vi "Init Plot Toolbar.vi"(7 "panel mode":T1, 8 "error in (no error)":errorcluster, 11 "Refs":T2) -> (0 "error out":errorcluster, 3 "Refs (dup)":T2)   [LabVIEW 2021, in "RocketPlot.lvlib"]
uses:
  RocketPlot.lvlib
  TypeDefs/Plot UI references.ctl
  <userlib>/bjustice/TipStripOOPanel/Classes/TipPanelHandle/TipPanelHandle.lvclass
  TypeDefs/Plot top row.ctl
  Classes/RocketPlotHandle/RocketPlotHandle.lvclass
  TypeDefs/panel mode.ctl
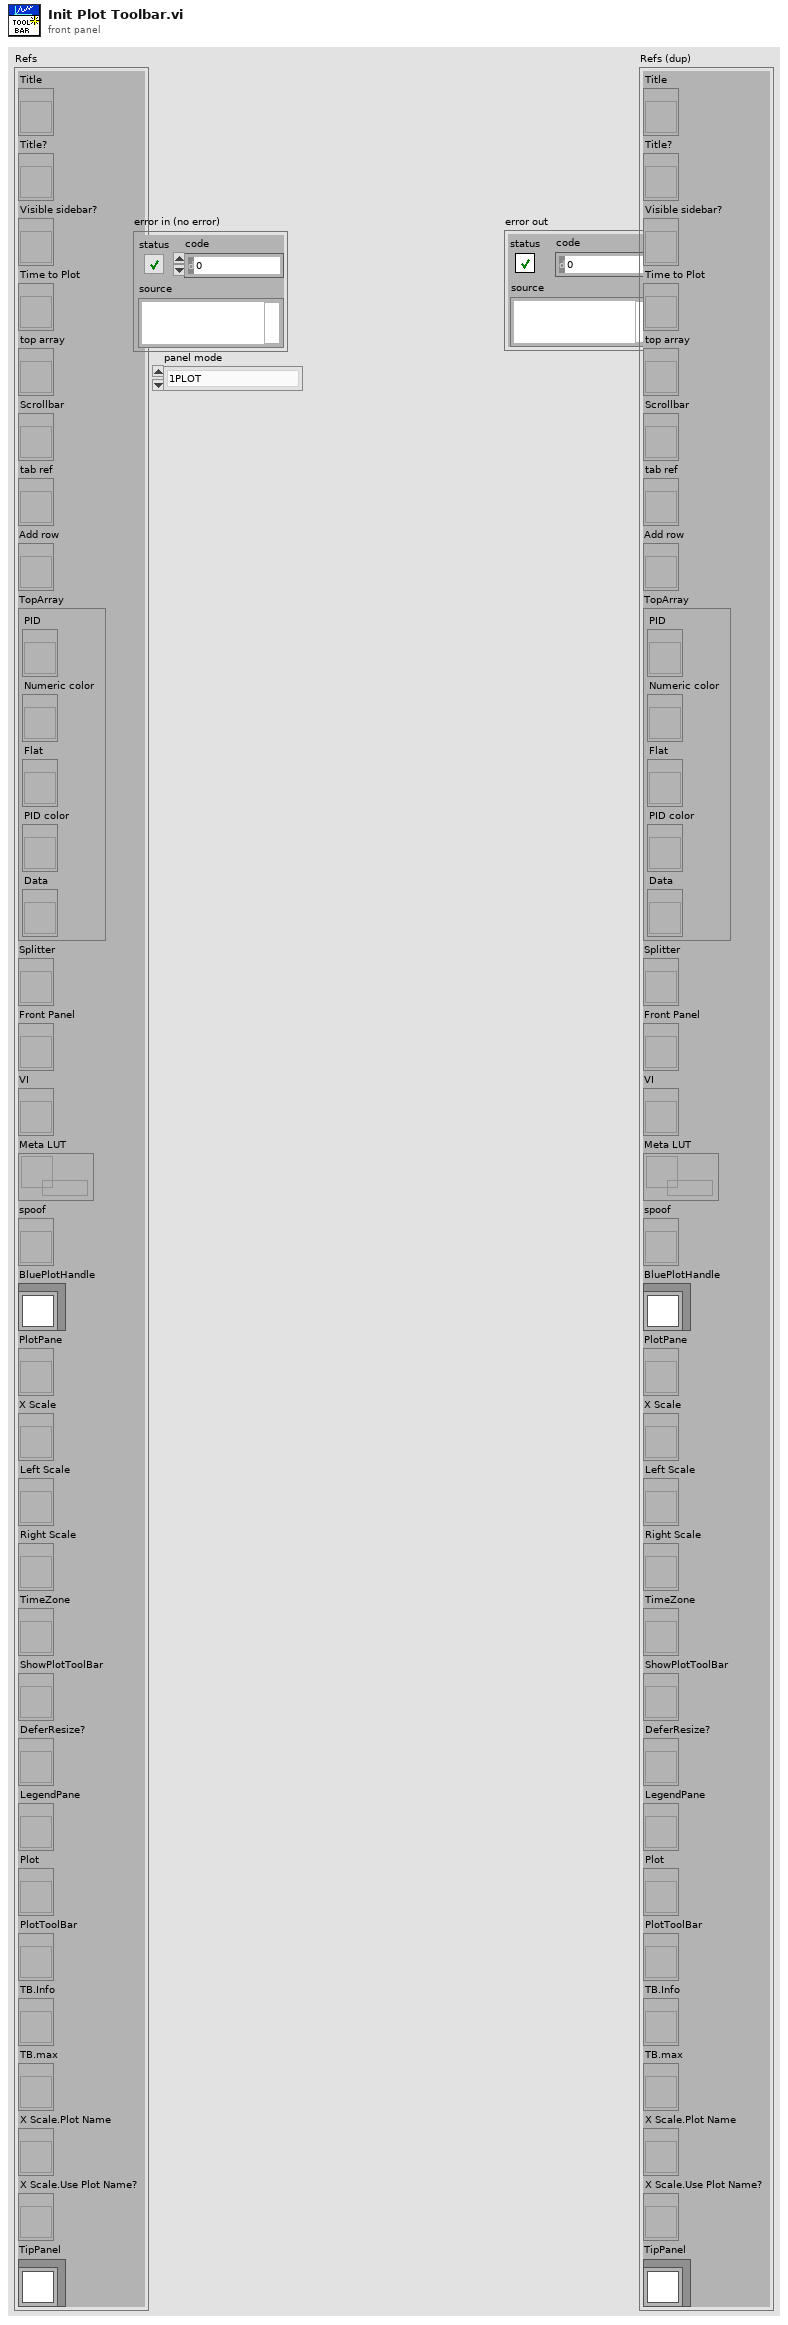
[diagram p1: front panel]
types:
  T1 = typedef "RocketPlot.lvlib/panel mode.ctl" = enum16{"1PLOT", "MPLOT"}
  T2 = typedef "RocketPlot.lvlib/Plot UI references.ctl" = cluster{"Title":refnum<vi>, "Title?":refnum<vi>, "Visible sidebar?":refnum<vi>, "Time to Plot":refnum<vi>, "top array":refnum<vi>, "Scrollbar":refnum<vi>, "tab ref":refnum<vi>, "Add row":refnum<vi>, "TopArray":cluster{"PID":refnum<vi>, "Numeric color":refnum<vi>, "Flat":refnum<vi>, "PID color":refnum<vi>, "Data":refnum<vi>}, "Splitter":refnum<vi>, "Front Panel":refnum<vi>, "VI":refnum<vi>, "Meta LUT":refnum<data-value>, "spoof":refnum<vi>, "BluePlotHandle":refnum<class "RocketPlotHandle.lvclass">, "PlotPane":refnum<vi>, "X Scale":refnum<vi>, "Left Scale":refnum<vi>, "Right Scale":refnum<vi>, "TimeZone":refnum<vi>, "ShowPlotToolBar":refnum<vi>, "DeferResize?":refnum<vi>, "LegendPane":refnum<vi>, "Plot":refnum<vi>, "PlotToolBar":refnum<vi>, "TB.Info":refnum<vi>, "TB.max":refnum<vi>, "X Scale.Plot Name":refnum<vi>, "X Scale.Use Plot Name?":refnum<vi>, "TipPanel":refnum<class "TipPanelHandle.lvclass">}
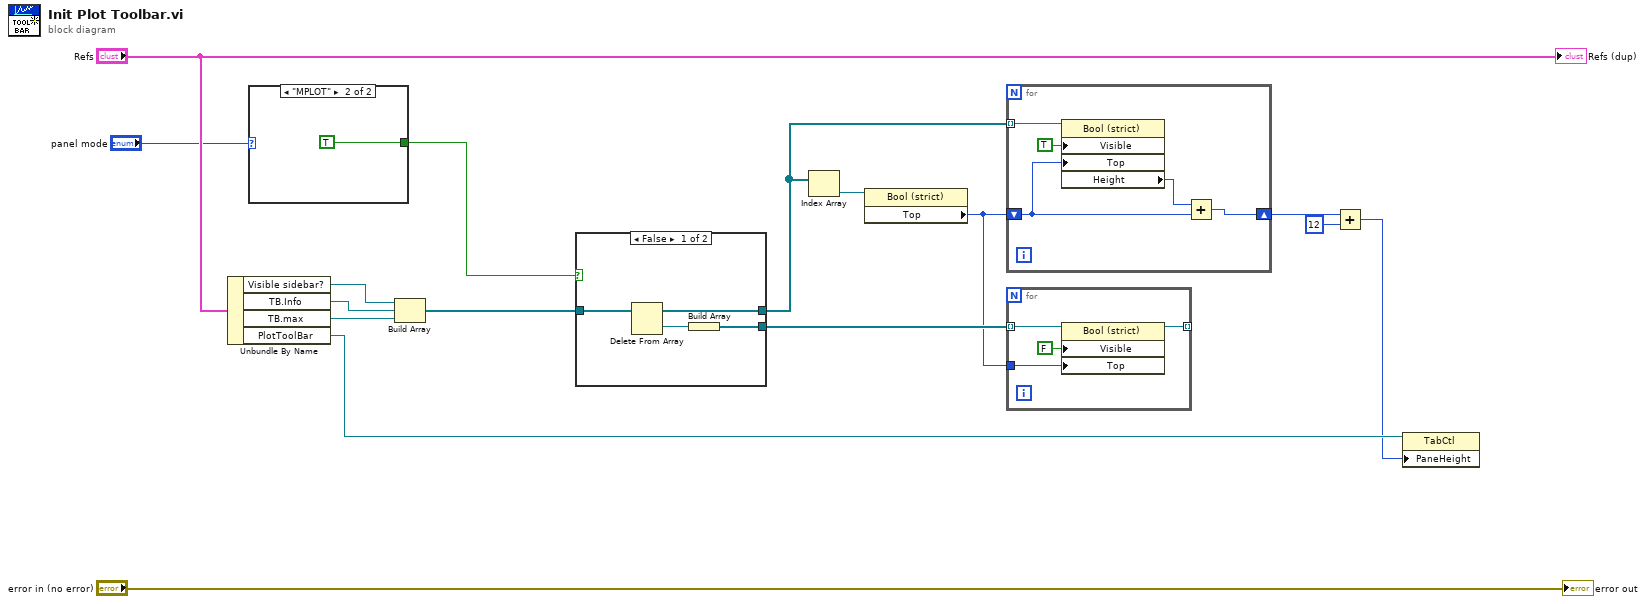
[diagram p0: block diagram]
diagram:
  n1 = Unbundle By Name("Refs") -> ("Visible sidebar?"=w15:refnum<vi>, "TB.Info"=w14:refnum<vi>, "TB.max"=w13:refnum<vi>, "PlotToolBar"=w6:refnum<vi>)
  n2 = case shown="\"MPLOT\"" "panel mode" {
    tunnel: [_ TRUE] -> w1
    frame "1PLOT" {
    }
    frame "MPLOT" {
    }
  }
  n3 = Build Array(w15, w14, w13) -> (w12:refnum<vi>[])
  n4 = case shown="False" w1 {
    tunnel: w12 -> [w21 w22]
    tunnel: [w19 w22] -> w9
    tunnel: [w18 _] -> w11
    frame False {
      n5 = Delete From Array(array=w21) -> (deleted portion=w20:refnum<vi>, array with subset deleted=w19:refnum<vi>[])  [unwired: 2 in]
      n6 = Build Array(w20) -> (w18:refnum<vi>[])
    }
    frame True {
    }
  }
  n7 = Index Array(array=w9) -> (element=w10:refnum<vi>)  [unwired: 1 in]
  n8 = property class="Bool (strict)"(reference=w10) -> ("Top"=w8:i32)  [unwired: 1 in, 2 out]
  n9 = for {
    tunnel: w9 -> [w27] mode=indexing
    shift-right: [w23] -> w4
    shift-left: w8 -> [w24]
    n10 = property class="Bool (strict)"(reference=w27, "Visible"=TRUE, "Top"=w24) -> ("Height"=w25:u32)  [unwired: 1 in, 2 out]
    n11 = Add(x=w25, y=w24) -> (x+y=w23:u32)
  }
  n12 = for {
    tunnel: w11 -> [w31] mode=indexing
    tunnel: w8 -> [w29]
    tunnel: [w28] -> _ mode=indexing
    n13 = property class="Bool (strict)"(reference=w31, "Visible"=FALSE, "Top"=w29) -> (reference out=w28:refnum<vi>)  [unwired: 1 in, 1 out]
  }
  n14 = Add(x=w4, y=u32 12) -> (x+y=w3:u32)
  n15 = property class="TabCtl"(reference=w6, "PaneHeight"=w3) -> ()  [unwired: 1 in, 2 out]
  "error out" <- "error in (no error)"
  "Refs (dup)" <- "Refs"
